vi "Set Turn Table Speed.vi"(8 "error in (no error)":errorcluster, 11 "CO3000 in":refnum<class "CO3000.lvclass">) -> (0 "error out":errorcluster, 3 "CO3000 out":refnum<class "CO3000.lvclass">)   [LabVIEW 2023, in "Turn Table and Mast.lvlib" / "CO3000.lvclass"]
uses:
  CO3000.lvclass
  CO3000.lvclass/CO3000.ctl
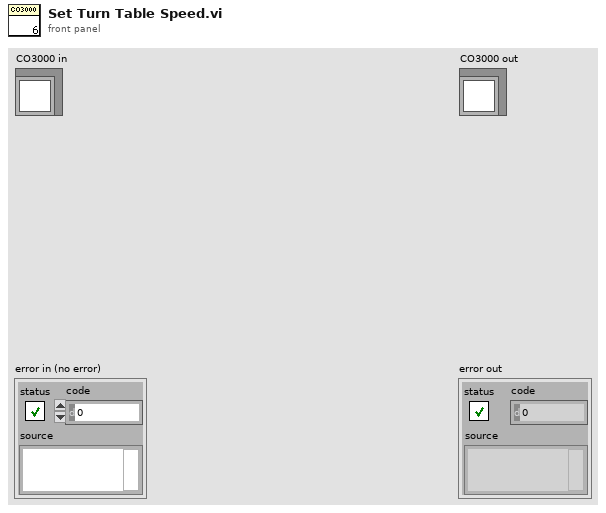
[diagram p1: front panel]
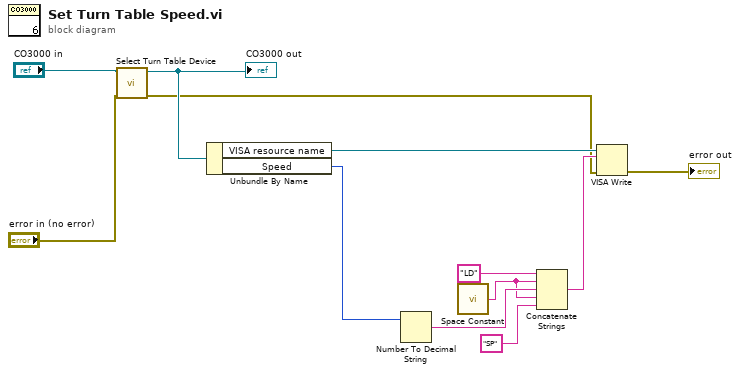
[diagram p0: block diagram]
diagram:
  n1 = call "Select Turn Table Device.vi"("error in (no error)"="error in (no error)", "CO3000 in"="CO3000 in") -> ("error out"=w2:errorcluster, "CO3000 out"=w3:refnum<class "CO3000.lvclass">)  [unwired: 8 in]
  "CO3000 out" <- w3
  n2 = Unbundle By Name(w3) -> ("VISA resource name"=w12:refnum<visa-resource-name>, "Speed"=w11:i32)
  n3 = Number To Decimal String(number=w11) -> (decimal integer string=w9:string)  [unwired: 1 in]
  n4 = call <vilib>:"Space Constant.vi"() -> ("String"=w8:string)
  n5 = Concatenate Strings("LD" ("string"), w8, w9, w8, "SP" ("string")) -> (w6:string)
  n6 = VISA Write(VISA resource name=w12, write buffer=w6, error in (no error)=w2) -> (error out=→"error out":errorcluster)  [unwired: 2 out]
